vi "VIH HelpGen - Image - Adapt Ctrl Name for Search in Conpane Picture.vi"(11 "name":string) -> (3 "Conpane name out":string)   [LabVIEW 2014]
doc: "::: VI Helpeks :::\nCopyright (c) 2000-2026 Konstantin Shifershteyn. All rights reserved."
panel:
  # "VI Helpeks\nCopyright (c) 2012-2026 Konstantin Shifershteyn"
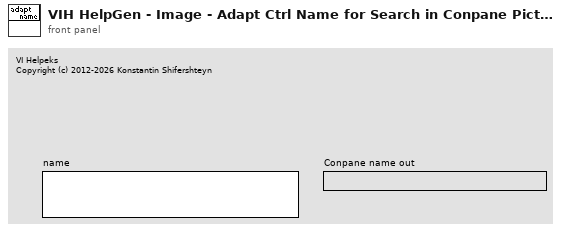
[diagram p1: front panel]
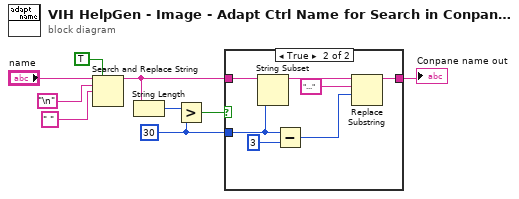
[diagram p0: block diagram]
diagram:
  w6 = 30 ("y")
  n1 = Search and Replace String(replace all?=TRUE, input string="name", search string="\n", replace string=" ") -> (result string=w1:string)  [unwired: 4 in, 3 out]
  n2 = String Length(string=w1) -> (length=w8:i32)
  n3 = Greater?(x=w8, y=w6) -> (0:w7:bool)
  n4 = case shown="True" w7 {
    tunnel: [w10 w17] -> w9
    tunnel: w1 -> [w10 w13]
    tunnel: w6 -> [_ w11]
    frame False {
    }
    frame True {
      n5 = String Subset(string=w13, length (rest)=w11) -> (substring=w12:string)  [unwired: 1 in]
      n6 = Subtract(x=w11, y=3) -> (x-y=w14:i32)
      n7 = Replace Substring(3:w14, 4:"..." ("substring (\"\")"), 5:w12) -> (1:w17:string)  [unwired: 1 in, 1 out]
    }
  }
  "Conpane name out" <- w9
